vi "CallBackVI.vi"(4 "User Parameter":variant, 5 "Event Data":cluster{"e":refnum<k24>}, 6 "Control Ref":refnum<k24>, 7 "Event Common Data":T1) -> ()   [LabVIEW 2026]
uses:
  C:/Users/loicw/Documents/LabVIEW/ToastNotifications/Sources/bins/Microsoft.Toolkit.Uwp.Notifications.dll
  bins/Microsoft.Toolkit.Uwp.Notifications.dll
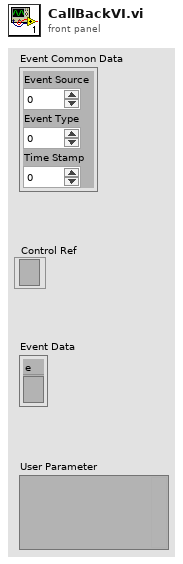
[diagram p1: front panel]
types:
  T1 = cluster{"Event Source":i32, "Event Type":u32, "Time Stamp":u32}
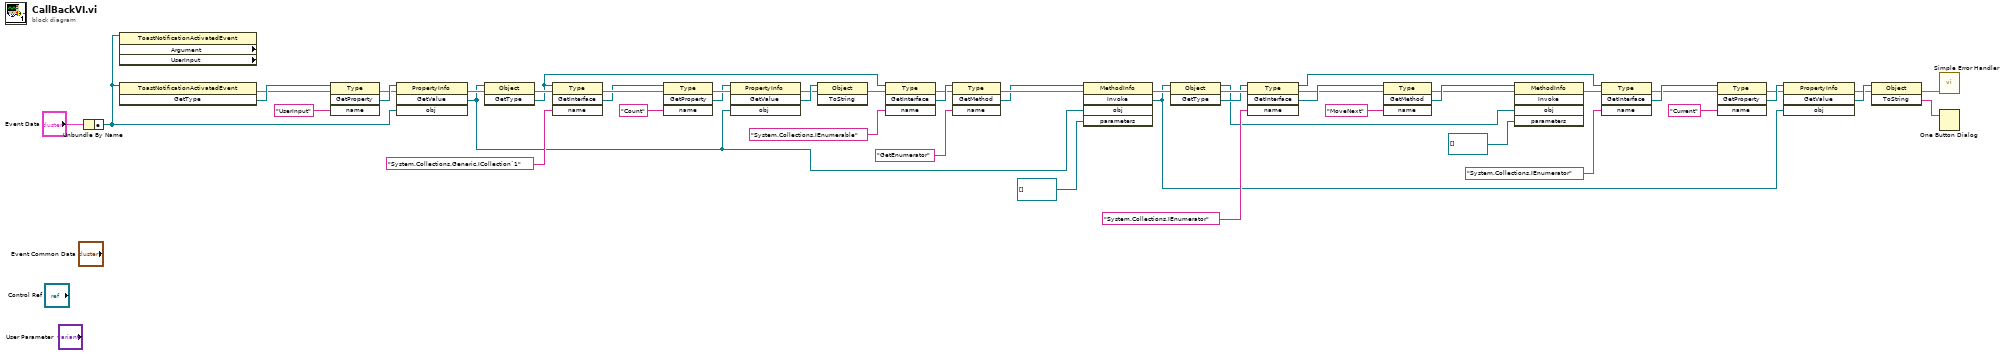
[diagram p0: block diagram]
diagram:
  n1 = Unbundle By Name("Event Data") -> ("e"=w48:refnum<k24>)
  n2 = property class="ToastNotificationActivatedEvent" props=["Argument", "UserInput"](reference=w48) -> ()  [unwired: 1 in, 4 out]
  n3 = invoke class="ToastNotificationActivatedEvent" method="GetType"(reference=w48) -> (error out=w46:errorcluster, "GetType"=w50:refnum<k24>)  [unwired: 2 in, 1 out]
  n4 = invoke class="Type" method="GetProperty"(reference=w50, error in=w46, "name"="UserInput") -> (error out=w45:errorcluster, "GetProperty"=w49:refnum<k24>)  [unwired: 1 in, 2 out]
  n5 = invoke class="PropertyInfo" method="GetValue"(reference=w49, error in=w45, "obj"=w48) -> (error out=w44:errorcluster, "GetValue"=w27:refnum<k24>)  [unwired: 1 in, 2 out]
  n6 = invoke class="Object" method="GetType"(reference=w27, error in=w44) -> (error out=w43:errorcluster, "GetType"=w33:refnum<k24>)  [unwired: 1 in, 1 out]
  n7 = invoke class="Type" method="GetInterface"(reference=w33, error in=w43, "name"="System.Collections.Generic.ICollection`1") -> (error out=w41:errorcluster, "GetInterface"=w40:refnum<k24>)  [unwired: 1 in, 2 out]
  n8 = invoke class="Type" method="GetProperty"(reference=w40, error in=w41, "name"="Count") -> (error out=w38:errorcluster, "GetProperty"=w37:refnum<k24>)  [unwired: 1 in, 2 out]
  n9 = invoke class="PropertyInfo" method="GetValue"(reference=w37, error in=w38, "obj"=w27) -> (error out=w35:errorcluster, "GetValue"=w36:refnum<k24>)  [unwired: 1 in, 2 out]
  n10 = invoke class="Object" method="ToString"(reference=w36, error in=w35) -> (error out=w32:errorcluster)  [unwired: 1 in, 2 out]
  n11 = invoke class="Type" method="GetInterface"(reference=w33, error in=w32, "name"="System.Collections.IEnumerable") -> (error out=w29:errorcluster, "GetInterface"=w31:refnum<k24>)  [unwired: 1 in, 2 out]
  n12 = invoke class="Type" method="GetMethod"(reference=w31, error in=w29, "name"="GetEnumerator") -> (error out=w28:errorcluster, "GetMethod"=w21:refnum<k24>)  [unwired: 1 in, 2 out]
  n13 = invoke class="MethodInfo" method="Invoke"(reference=w21, error in=w28, "obj"=w27, "parameters"=refnum<k24>[] []) -> (error out=w25:errorcluster, "Invoke"=w5:refnum<k24>)  [unwired: 1 in, 3 out]
  n14 = invoke class="Object" method="GetType"(reference=w5, error in=w25) -> (reference out=w7:refnum<k24>, error out=w18:errorcluster, "GetType"=w14:refnum<k24>)  [unwired: 1 in]
  n15 = invoke class="Type" method="GetInterface"(reference=w14, error in=w18, "name"="System.Collections.IEnumerator") -> (reference out=w6:refnum<k24>, error out=w17:errorcluster, "GetInterface"=w23:refnum<k24>)  [unwired: 1 in, 1 out]
  n16 = invoke class="Type" method="GetMethod"(reference=w23, error in=w17, "name"="MoveNext") -> (error out=w16:errorcluster, "GetMethod"=w20:refnum<k24>)  [unwired: 1 in, 2 out]
  n17 = invoke class="MethodInfo" method="Invoke"(reference=w20, error in=w16, "obj"=w7, "parameters"=refnum<k24>[] []) -> (error out=w15:errorcluster)  [unwired: 1 in, 4 out]
  n18 = invoke class="Type" method="GetInterface"(reference=w6, error in=w15, "name"="System.Collections.IEnumerator") -> (error out=w9:errorcluster, "GetInterface"=w12:refnum<k24>)  [unwired: 1 in, 2 out]
  n19 = invoke class="Type" method="GetProperty"(reference=w12, error in=w9, "name"="Current") -> (error out=w8:errorcluster, "GetProperty"=w10:refnum<k24>)  [unwired: 1 in, 2 out]
  n20 = invoke class="PropertyInfo" method="GetValue"(reference=w10, error in=w8, "obj"=w5) -> (error out=w3:errorcluster, "GetValue"=w4:refnum<k24>)  [unwired: 1 in, 2 out]
  n21 = invoke class="Object" method="ToString"(reference=w4, error in=w3) -> (error out=w1:errorcluster, "ToString"=w2:string)  [unwired: 1 in, 1 out]
  n22 = call <vilib>:"Simple Error Handler.vi"("error in (no error)"=w1) -> ()  [unwired: 4 in, 5 out]
  n23 = One Button Dialog(message=w2) -> ()  [unwired: 1 in, 1 out]
